vi "Get Object Type.vi"(8 "error in (no error)":errorcluster, 11 "Object in":refnum<k24>) -> (0 "error out":errorcluster, 2 "Object Type":refnum<k24>, 3 "Object out":refnum<k24>)   [LabVIEW 2026, in "ToastNotification.lvlib" / "Reflection DotNet.lvlib"]
doc: "Native Object.GetType call. Borrow Object in and acquire its runtime System.Type handle as Object Type. Object out aliases the input object. Caller closes Object Type after reflection work, including on an error path; this VI does not close Object in."
uses:
  Reflection DotNet.lvlib
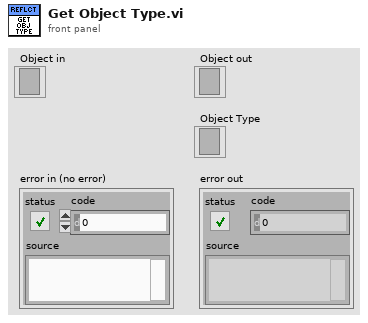
[diagram p1: front panel]
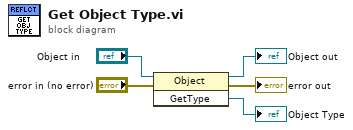
[diagram p0: block diagram]
diagram:
  n1 = invoke class="Object" method="GetType"(reference="Object in", error in="error in (no error)") -> (reference out=→"Object out":refnum<k24>, error out=→"error out":errorcluster, "GetType"=→"Object Type":refnum<k24>)  [unwired: 1 in]
